vi "Get Status.vi"(8 "error in":errorcluster, 11 "GUID":string) -> (0 "error out":errorcluster, 3 "Messages":i32)   [LabVIEW 2025, in "CAN-LIN Raw Bus Capture.lvclass"]
uses:
  CAN-LIN Raw Bus Capture.lvclass
  CAN-LIN Raw Bus Capture.lvclass/CAN-LIN Raw Bus Capture.ctl
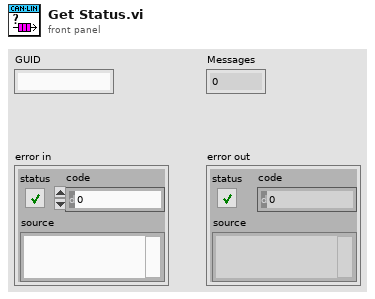
[diagram p1: front panel]
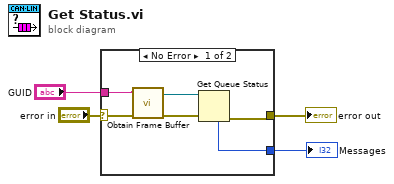
[diagram p0: block diagram]
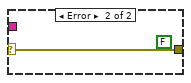
[diagram p2: hidden frame]
diagram:
  n1 = case shown="No Error" "error in" {
    selector: "error in" -> [w10 w11]
    tunnel: [w7 w11] -> w3
    tunnel: [w6 _] -> w2
    tunnel: "GUID" -> [w5 _]
    frame No Error {
      n2 = call "Obtain Frame Buffer.vi"("error in"=w10, "GUID"=w5) -> ("error out"=w8:errorcluster, "queue out"=w9:refnum<queue>)  [unwired: 8 in]
      n3 = Get Queue Status(queue=w9, error in (no error)=w8) -> (error out=w7:errorcluster, # elements in queue=w6:i32)  [unwired: 1 in, 6 out]
    }
    frame Error {
      (unwired) FALSE ("overflow?")
    }
  }
  "error out" <- w3
  "Messages" <- w2
